vi "Set Item.vi"(8 "error in (no error)":errorcluster, 9 "JSON Scalar":refnum<class "JSON Scalar.lvclass">, 10 "Name":string, 11 "json class in":refnum<class "json class.lvclass">) -> (0 "error out":errorcluster, 3 "json class out":refnum<class "json class.lvclass">)   [LabVIEW 2021, in "Config Library.lvlib" / "json class.lvclass"]
uses:
  json class.lvclass
  <vilib>/addons/JSON API/JSON Scalar/JSON Scalar.lvclass
  C:/Program Files (x86)/National Instruments/LabVIEW 2021/vi.lib/addons/JSON API/JSON Value/JSON Value.lvclass
  json class.lvclass/json class.ctl
  <vilib>/addons/JSON API/JSON Object/Set Object Item by name.vi
  <vilib>/addons/JSON API/JSON Object/JSON Object.lvclass
  <vilib>/addons/JSON API/Get Polymorphic/JSON GetSet.lvlib
  C:/Program Files (x86)/National Instruments/LabVIEW 2021/vi.lib/addons/JSON API/JSON Scalar/JSON Scalar.lvclass
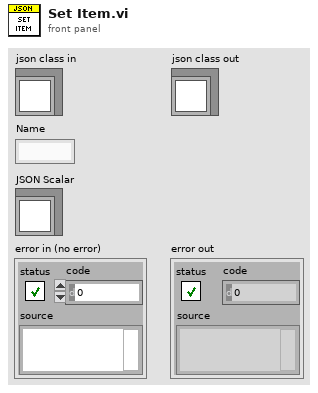
[diagram p1: front panel]
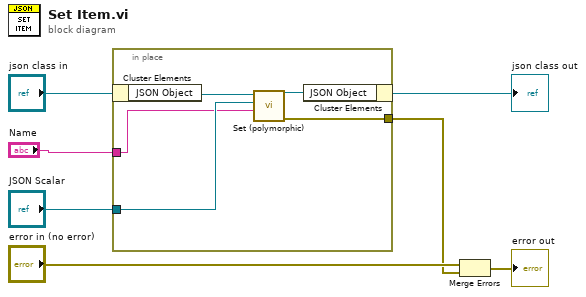
[diagram p0: block diagram]
diagram:
  n1 = in-place {
    in-place-border: [w10] -> w3
    in-place-border: "JSON Scalar" -> [w9]
    in-place-border: "Name" -> [w8]
    n2 = in-place-cluster #1("json class in") -> ("JSON Object"=w11:refnum<class "JSON Object.lvclass">)
    n3 = call-poly <vilib>:"Set (polymorphic).vi"("name"=w8, "Value"=w9, "JSON Object in"=w11) -> ("error out"=w10:errorcluster, "JSON Object out"=w12:refnum<class "JSON Object.lvclass">)  [unwired: 6 in, 1 out]
    n4 = in-place-cluster #1("JSON Object"=w12) -> (→"json class out":refnum<class "json class.lvclass">)
  }
  n5 = Merge Errors("error in (no error)", w3) -> (→"error out":errorcluster)
